vi "onDestroy.vi"(8 "error in (no error)":errorcluster, 11 "MQTT_Base in":refnum<class "MQTT_Base.lvclass">) -> (0 "error out":errorcluster, 3 "MQTT_Base out":refnum<class "MQTT_Base.lvclass">)   [LabVIEW 2013, in "MQTT Base.lvlib" / "MQTT_Base.lvclass"]
uses:
  MQTT_Base.lvclass
  MQTT_Base.lvclass/MQTT_Base.ctl
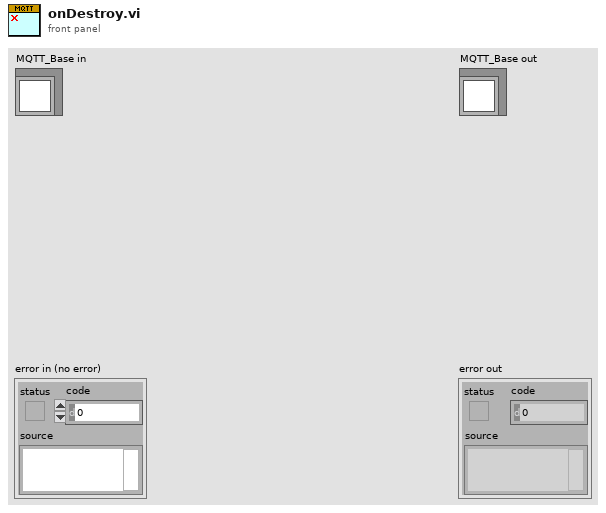
[diagram p1: front panel]
types:
  T1 = typedef "MQTT Base.lvlib/MQTT_Base.lvclass/Public Events -- cluster.ctl" = cluster{"Stop Event":refnum<user-event>, "Error Event":refnum<user-event>, "Inbound Message":refnum<user-event>}
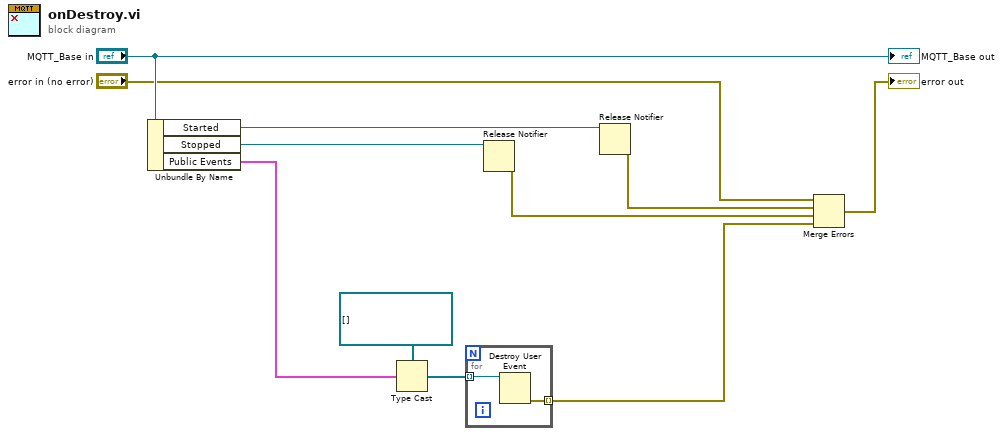
[diagram p0: block diagram]
diagram:
  n1 = Unbundle By Name("MQTT_Base in") -> ("Started"=w8:refnum<notifier>, "Stopped"=w9:refnum<notifier>, "Public Events"=w3:T1)
  n2 = Type Cast(type=refnum<user-event>[] [], x=w3) -> (*(type *) &x=w2:refnum<user-event>[])
  n3 = for {
    tunnel: w2 -> [w13] mode=indexing
    tunnel: [w12] -> w1 mode=indexing
    n4 = Destroy User Event(user event=w13) -> (error out=w12:errorcluster)  [unwired: 1 in]
  }
  n5 = Release Notifier(notifier=w9) -> (error out=w11:errorcluster)  [unwired: 2 in, 2 out]
  n6 = Release Notifier(notifier=w8) -> (error out=w10:errorcluster)  [unwired: 2 in, 2 out]
  n7 = Merge Errors("error in (no error)", w10, w11, w1) -> (→"error out":errorcluster)
  "MQTT_Base out" <- "MQTT_Base in"
